vi "RemoteVI Note Popup Pointer.vi"(0 "popup?":bool, 1 "geo":T1, 5 "msg":u32, 7 "x":i32, 9 "y":i32) -> ()   [LabVIEW 2020, in "RemoteVI.lvlib"]
doc: "Remembers the remote pointer while a LabVIEW popup is open (docs\\architecture.md, Popups): for a WM_MOUSEMOVE (512) with popup? TRUE the menu pointer state (RemoteVI Menu Pointer.vi) gets active TRUE, x, y = the LOGICAL screen point (frame origin geo.panelX, panelY + x, y - the frame is the window below its title bar), moved = now and navigated FALSE. Nothing is posted - a posted move does not move LabVIEW's menu highlight (it follows the real cursor); RemoteVI Menu Hover.vi applies the latest position with keys once per server loop iteration, so a burst of moves costs one navigation. Anything else does nothing. Pure G apart from the state."
uses:
  RemoteVI.lvlib
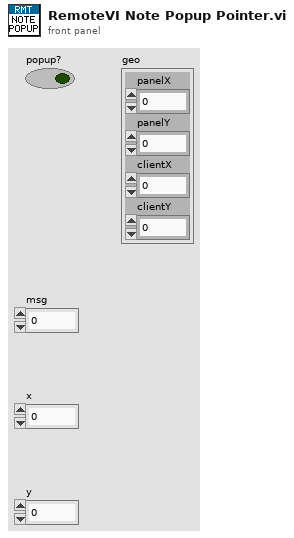
[diagram p1: front panel]
types:
  T1 = cluster{"panelX":i32, "panelY":i32, "clientX":i32, "clientY":i32}
  T2 = cluster{"active":bool, "x":i32, "y":i32, "moved":u32, "navigated":bool, "menu":u64, "top":i32, "hit":bool, "row since":u32, "dwelled":bool, "plain":u64, "swallow up":bool}
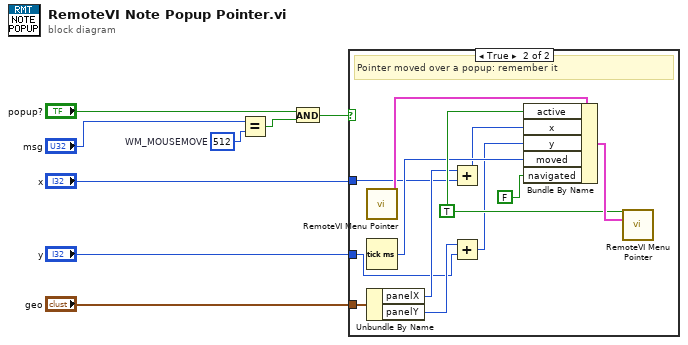
[diagram p0: block diagram]
diagram:
  w6 = u32 512  # WM_MOUSEMOVE
  n1 = Equal?(x="msg", y=w6) -> (x = y?=w7:bool)
  n2 = And(x="popup?", y=w7) -> (x .and. y?=w8:bool)
  n3 = case shown="True" w8 {
    tunnel: "x" -> [_ w9]
    tunnel: "y" -> [_ w10]
    tunnel: "geo" -> [_ w11]
    frame False {
    }
    frame True {
      w18 = TRUE
      # "Pointer moved over a popup: remember it"
      n4 = call "RemoteVI Menu Pointer.vi"() -> ("state"=w17:T2)  [unwired: 15 in]
      n5 = Tick Count (ms)() -> (millisecond timer value=w16:u32)
      n6 = Unbundle By Name(w11) -> ("panelX"=w12:i32, "panelY"=w13:i32)
      n7 = Add(x=w12, y=w9) -> (x+y=w14:i32)
      n8 = Add(x=w13, y=w10) -> (x+y=w15:i32)
      n9 = Bundle By Name(cluster=w17, "active"=w18, "x"=w14, "y"=w15, "moved"=w16, "navigated"=FALSE) -> (w20:T2)
      n10 = call "RemoteVI Menu Pointer.vi"("write?"=w18, "state in"=w20) -> ()  [unwired: 13 in, 1 out]
    }
  }
